vi "New Batch.vi"(6 "Batch ID":u32, 8 "error in (no error)":errorcluster, 9 "Buffer size":u32, 10 "OD Vars":T1[](array[typedef]) {"CANOpen Types" items=["bool"=1, "i8"=2, "i16"=3, "i32"=4, "u8"=5, "u16"=6, "u32"=7, "f32"=8, "visible str"=9, "octet str"=10, "f64"=17, "i64"=21, "u64"=27]; "OD Index"."SubIndex" format="%.0x"; "OD Index"."Index" format="%.0x"}, 11 "OD Batch in":refnum<class "OD Batch.lvclass">) -> (0 "error out":errorcluster, 3 "OD Batch out":refnum<class "OD Batch.lvclass">)   [LabVIEW 2023, in "xnet_canopen.lvlib" / "OD Batch.lvclass"]
uses:
  OD Batch.lvclass
  OD Batch.lvclass/OD Batch.ctl
  typedef/od index.ctl
  xnet_canopen.lvlib
  typedef/canopen types.ctl
  typedef/od entry.ctl
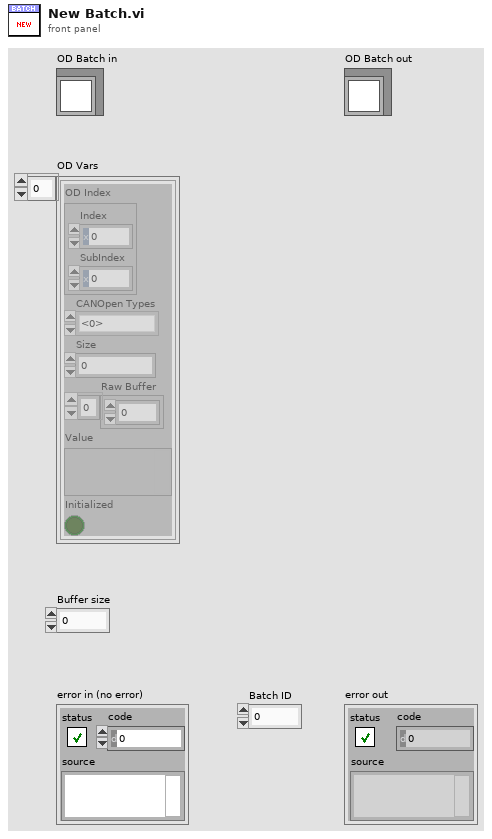
[diagram p1: front panel]
types:
  T1 = typedef "xnet_canopen.lvlib/od entry.ctl" = cluster{"OD Index":T2, "CANOpen Types":T3, "Size":u32, "Raw Buffer":u8[], "Value":variant, "Initialized":bool}
  T2 = typedef "xnet_canopen.lvlib/od index.ctl" = cluster{"Index":u16, "SubIndex":u8}
  T3 = typedef "xnet_canopen.lvlib/canopen types.ctl" = u32
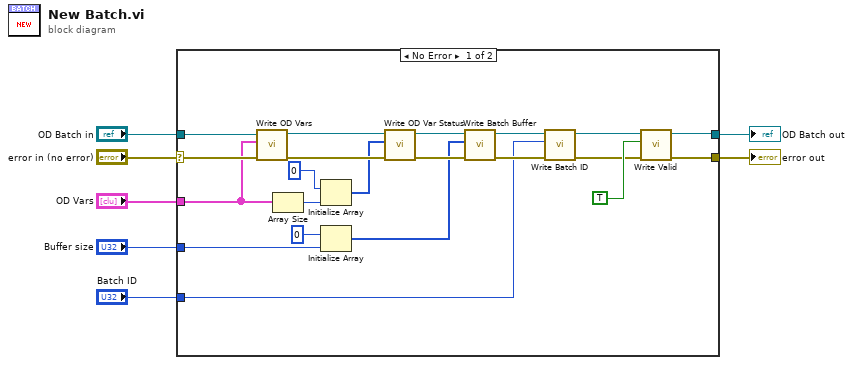
[diagram p0: block diagram]
diagram:
  n1 = case shown="No Error" "error in (no error)" {
    selector: "error in (no error)" -> [w22 w30]
    tunnel: [w21 w30] -> w6
    tunnel: [w19 w29] -> w4
    tunnel: "OD Batch in" -> [w20 w29]
    tunnel: "OD Vars" -> [w15 _]
    tunnel: "Buffer size" -> [w10 _]
    tunnel: "Batch ID" -> [w8 _]
    frame No Error {
      n2 = call "Write OD Vars.vi"("error in (no error)"=w22, "OD Vars"=w15, "OD Batch in"=w20) -> ("error out"=w27:errorcluster, "OD Batch out"=w17:refnum<class "OD Batch.lvclass">)  [unwired: 7 in]
      n3 = Array Size(array=w15) -> (size(s)=w14:i32)
      n4 = Initialize Array(0 ("element"), w14) -> (w12:i32[])
      n5 = Initialize Array(u8 0 ("element"), w10) -> (w11:u8[])
      n6 = call "Write OD Var Status.vi"("error in (no error)"=w27, "OD Var Status"=w12, "OD Batch in"=w17) -> ("error out"=w18:errorcluster, "OD Batch out"=w16:refnum<class "OD Batch.lvclass">)  [unwired: 7 in]
      n7 = call "Write Batch Buffer.vi"("error in (no error)"=w18, "Batch Buffer"=w11, "OD Batch in"=w16) -> ("error out"=w24:errorcluster, "OD Batch out"=w28:refnum<class "OD Batch.lvclass">)  [unwired: 7 in]
      n8 = call "Write Batch ID.vi"("error in (no error)"=w24, "Batch ID"=w8, "OD Batch in"=w28) -> ("error out"=w23:errorcluster, "OD Batch out"=w26:refnum<class "OD Batch.lvclass">)  [unwired: 7 in]
      n9 = call "Write Valid.vi"("error in (no error)"=w23, "Valid"=TRUE, "OD Batch in"=w26) -> ("error out"=w21:errorcluster, "OD Batch out"=w19:refnum<class "OD Batch.lvclass">)  [unwired: 7 in]
    }
    frame Error {
    }
  }
  "error out" <- w6
  "OD Batch out" <- w4
